vi "SeqEditor_StepMLST-ReNameBox.vi"(8 "error in (no error)":errorcluster, 11 "NLTest in":refnum<class "NLTest.lvclass">) -> (0 "error out":errorcluster, 3 "NLTest out":refnum<class "NLTest.lvclass">)   [LabVIEW 2017, in "NLTest.lvclass"]
uses:
  NLTest.lvclass
  <vilib>/Utility/miscctls.llb/LVRowAndColumnTypeDef.ctl
  VISTEP.ctl
  VISTEP_class_INOUTPUT.ctl
  VISTEP_class_INOUTPUT_TYPE.ctl
  NLTest.lvclass/NLTest.ctl
  SeqEditor_Global.vi
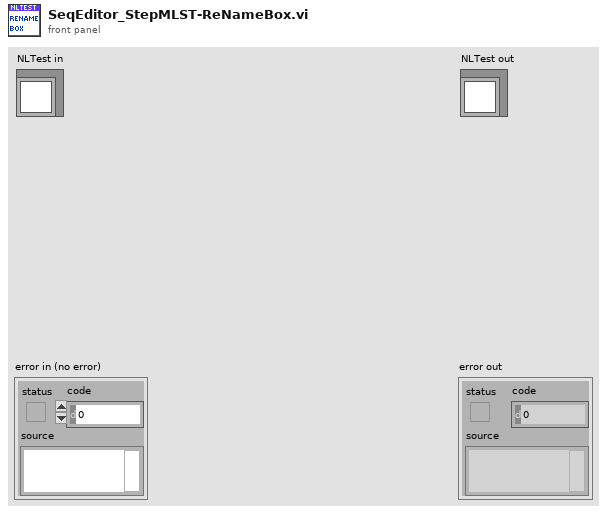
[diagram p1: front panel]
types:
  T1 = typedef "NLTest.lvclass/VISTEP.ctl" = cluster{"My":cluster{"VIpath":T2, "VIname":T2, "Loop":T2, "Skip":T2, "FailStop":T2, "StepClass":T2, "StringTest-Source":T2, "StringTest-Lim":T2, "BoolTest-Source":T2, "BoolTest-Lim":T2, "NumberTest-OP":T2, "NumberTest-Source":T2, "NumberTest-LimA":T2, "NumberTest-LimB":T2}, "INPUT":T2[], "OUTPUT":T2[]}
  T2 = typedef "NLTest.lvclass/VISTEP_class_INOUTPUT.ctl" = cluster{"ITEM":string, "DATA":string, "TYPE":T3, "TYPEDATA":string, "SV":bool, "clusterchain":refnum<vi>[]}
  T3 = typedef "NLTest.lvclass/VISTEP_class_INOUTPUT_TYPE.ctl" = enum16{"Number", "String", "Bool", "Enum", "Path", "VISA", "NA"}
  T4 = typedef "LVRowAndColumnTypeDef.ctl" = cluster{"Row":i32, "Column":i32}
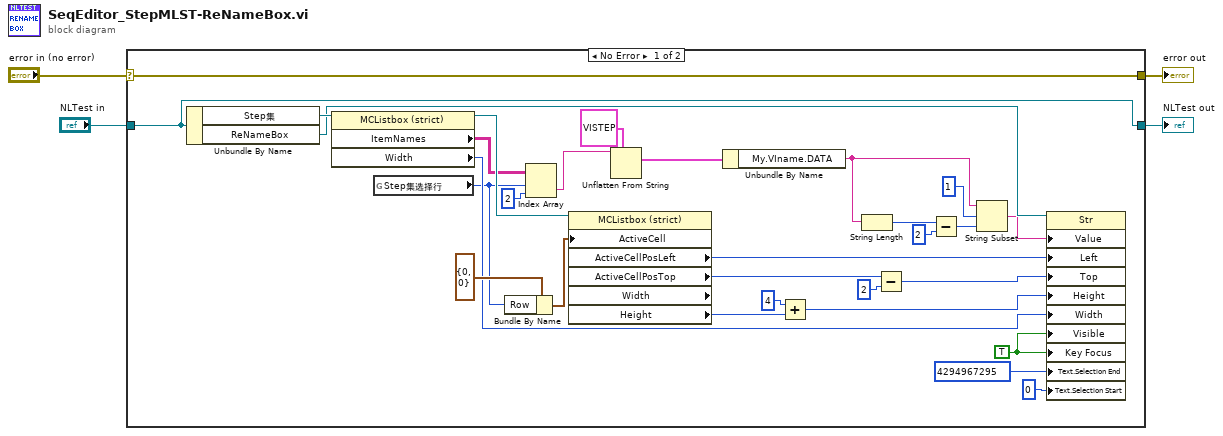
[diagram p0: block diagram]
diagram:
  n1 = case shown="No Error" "error in (no error)" {
    selector: "error in (no error)" -> [w34 w36]
    tunnel: [w34 w36] -> w3
    tunnel: [w33 w35] -> w1
    tunnel: "NLTest in" -> [w33 w35]
    frame No Error {
      w24 = TRUE ("Visible")
      n2 = Unbundle By Name(w33) -> ("Step集"=w31:refnum<vi>, "ReNameBox"=w29:refnum<vi>)
      n3 = property class="MCListbox (strict)"(reference=w31) -> (reference out=w25:refnum<vi>, "ItemNames"=w23:string[][], "Width"=w6:u32)  [unwired: 1 in, 1 out]
      n4 = global read "SeqEditor_Global.vi" "Step集选择行"() -> (w5:i32)
      n5 = Bundle By Name(cluster=T4 {"Row"=0, "Column"=0} ("Active Cell:Active Cell"), "Row"=w5) -> (w30:T4)
      n6 = Index Array(array=w23, index (row)=w5, index (col)=2 ("disabled index (col)")) -> (element=w20:string)
      n7 = property class="MCListbox (strict)" props=["ActiveCell", "ActiveCellPosLeft", "ActiveCellPosTop", "Width", "Height"](reference=w25, "ActiveCell"=w30) -> ("ActiveCellPosLeft"=w28:i32, "ActiveCellPosTop"=w27:i32, "Height"=w26:u32)  [unwired: 1 in, 3 out]
      n8 = Unflatten From String(type=T1 {"My"={"VIpath"={"ITEM"="VI路径", "DATA"="\"\"", "TYPE"=enum."Path", "TYPEDATA"="", "SV"=FALSE, "clusterchain"=[]}, "VIname"={"ITEM"="步骤名称", "DATA"="\"\"", "TYPE"=enum."String", "TYPEDATA"="", "SV"=FALSE, "clusterchain"=[]}, "Loop"={"ITEM"="重测次数", "DATA"="1", "TYPE"=enum."Number", "TYPEDATA"="", "SV"=FALSE, "clusterchain"=[]}, "Skip"={"ITEM"="跳过步骤", "DATA"="FALSE", "TYPE"=enum."Bool", "TYPEDATA"="", "SV"=FALSE, "clusterchain"=[]}, "FailStop"={"ITEM"="失败停止", "DATA"="FALSE", "TYPE"=enum."Bool", "TYPEDATA"="", "SV"=FALSE, "clusterchain"=[]}, "StepClass"={"ITEM"="步骤类型", "DATA"="NotaTEST", "TYPE"=enum."Enum", "TYPEDATA"="", "SV"=FALSE, "clusterchain"=[]}, "StringTest-Source"={"ITEM"="字符串测试值", "DATA"="\"\"", "TYPE"=enum."String", "TYPEDATA"="", "SV"=FALSE, "clusterchain"=[]}, "StringTest-Lim"={"ITEM"="字符串测试门限", "DATA"="\"\"", "TYPE"=enum."String", "TYPEDATA"="", "SV"=FALSE, "clusterchain"=[]}, "BoolTest-Source"={"ITEM"="布尔测试值", "DATA"="TRUE", "TYPE"=enum."Bool", "TYPEDATA"="", "SV"=FALSE, "clusterchain"=[]}, "BoolTest-Lim"={"ITEM"="布尔测试门限", "DATA"="TRUE", "TYPE"=enum."Bool", "TYPEDATA"="", "SV"=FALSE, "clusterchain"=[]}, "NumberTest-OP"={"ITEM"="数值测试OP", "DATA"="NotaTEST", "TYPE"=enum."Enum", "TYPEDATA"="", "SV"=FALSE, "clusterchain"=[]}, "NumberTest-Source"={"ITEM"="数值测试值", "DATA"="0", "TYPE"=enum."Number", "TYPEDATA"="", "SV"=FALSE, "clusterchain"=[]}, "NumberTest-LimA"={"ITEM"="数值测试门限A", "DATA"="0", "TYPE"=enum."Number", "TYPEDATA"="", "SV"=FALSE, "clusterchain"=[]}, "NumberTest-LimB"={"ITEM"="数值测试门限B", "DATA"="0", "TYPE"=enum."Number", "TYPEDATA"="", "SV"=FALSE, "clusterchain"=[]}}, "INPUT"=[], "OUTPUT"=[]} ("步骤结构"), binary string=w20) -> (value=w19:T1)  [unwired: 3 in, 2 out]
      n9 = Unbundle By Name(w19) -> ("My.VIname.DATA"=w16:string)
      n10 = Add(x=u32 4, y=w26) -> (x+y=w10:u32)
      n11 = String Length(string=w16) -> (length=w18:i32)
      n12 = Subtract(x=w27, y=2 ("x")) -> (x-y=w8:i32)
      n13 = Subtract(x=w18, y=2) -> (x-y=w14:i32)
      n14 = String Subset(string=w16, offset (0)=1, length (rest)=w14) -> (substring=w13:string)
      n15 = property class="Str"(reference=w29, "Value"=w13, "Left"=w28, "Top"=w8, "Height"=w10, "Width"=w6, "Visible"=w24, "Key Focus"=w24, "Text.Selection End"=u32 4294967295 ("Text.Selection:End"), "Text.Selection Start"=u32 0 ("Text.Selection:End")) -> ()  [unwired: 1 in, 2 out]
    }
    frame Error {
    }
  }
  "error out" <- w3
  "NLTest out" <- w1
